vi "Read configuration.vi"(8 "error in (no error)":errorcluster, 11 "Instrument Device in":refnum<class "PAC Instrument.lvclass">) -> (0 "error out":errorcluster, 2 "configuration":refnum<class "CEF_serializable configuration.lvclass">, 3 "Instrument Device out":refnum<class "PAC Instrument.lvclass">)   [LabVIEW 2025, in "PAC.lvlib" / "PAC Instrument.lvclass"]
uses:
  PAC Instrument.lvclass
  PAC Instrument.lvclass/PAC Instrument.ctl
  PAC configuration/PAC configuration.lvclass
  Users/Public/Documents/Sandia National Labs/TSS Plugin/CEF.lvlibp/serializable configuration/CEF_serializable configuration.lvclass
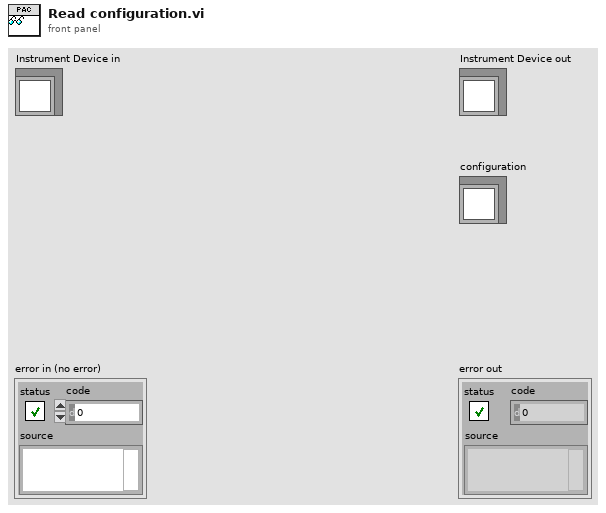
[diagram p1: front panel]
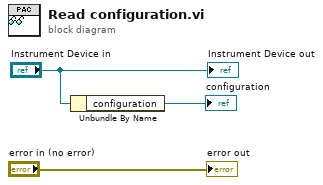
[diagram p0: block diagram]
diagram:
  n1 = Unbundle By Name("Instrument Device in") -> ("configuration"=→"configuration":refnum<class "PAC configuration.lvclass">)
  "error out" <- "error in (no error)"
  "Instrument Device out" <- "Instrument Device in"
